vi "VIH HelpGen - Get Control Info - Prepare Name & Description.vi"(9 "Description":string, 11 "Name":string) -> (1 "Description out":string, 3 "Name out":string)   [LabVIEW 2014]
doc: "::: VI Helpeks :::\nCopyright (c) 2000-2026 Konstantin Shifershteyn. All rights reserved."
panel:
  # "VI Helpeks\nCopyright (c) 2012-2026 Konstantin Shifershteyn"
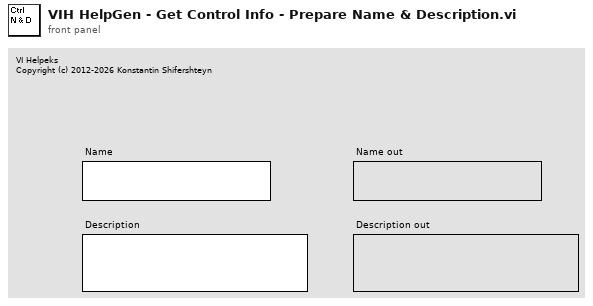
[diagram p1: front panel]
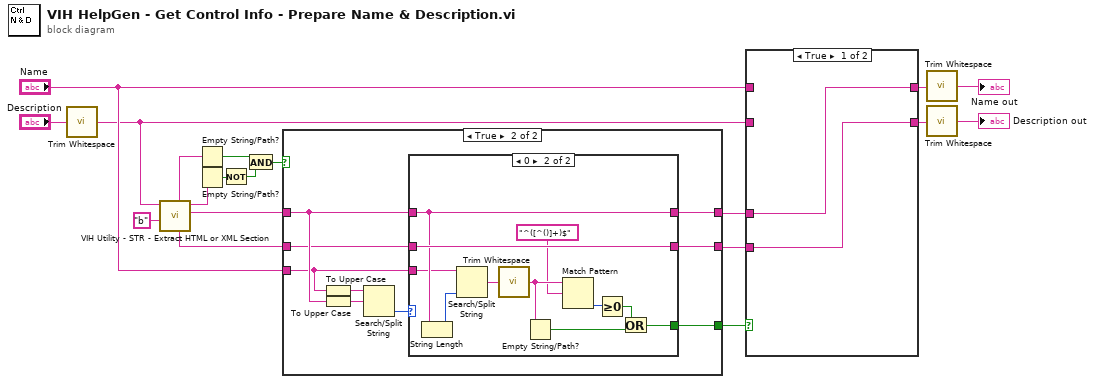
[diagram p0: block diagram]
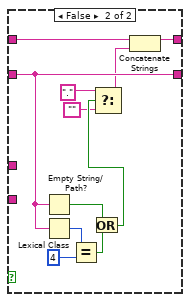
[diagram p2: hidden frame]
diagram:
  n1 = call <vilib>:"Trim Whitespace.vi"("string"="Description") -> ("trimmed string"=w3:string)  [unwired: 1 in]
  n2 = call "VIH Utility - STR - Extract HTML or XML Section.vi"("Section name"="b", "HTML in"=w3) -> ("body"=w11:string, "start"=w14:string, "after"=w10:string, "before"=w17:string)  [unwired: 5 in, 1 out]
  n3 = Empty String/Path?(string/path=w17) -> (empty?=w18:bool)
  n4 = Empty String/Path?(string/path=w14) -> (empty?=w13:bool)
  n5 = Not(x=w13) -> (.not. x?=w12:bool)
  n6 = And(x=w18, y=w12) -> (x .and. y?=w15:bool)
  n7 = case shown="True" w15 {
    tunnel: w11 -> [_ w25]
    tunnel: "Name" -> [_ w21]
    tunnel: [_ w24] -> w7
    tunnel: w10 -> [_ w23]
    tunnel: [_ w22] -> w2
    tunnel: [_ w20] -> w1
    frame False {
    }
    frame True {
      n8 = To Upper Case(1:w21) -> (0:w28:string)
      n9 = To Upper Case(1:w25) -> (0:w27:string)
      n10 = Search/Split String(string=w28, search string/char (-)=w27) -> (offset of match=w26:i32)  [unwired: 1 in, 2 out]
      n11 = case shown="0" w26 {
        tunnel: [_ w38] -> w24
        tunnel: w25 -> [_ w38]
        tunnel: w23 -> [_ w39]
        tunnel: [_ w39] -> w22
        tunnel: w21 -> [_ w37]
        tunnel: [_ w31] -> w20
        frame ..-1, Default {
        }
        frame 0 {
          n12 = String Length(string=w38) -> (length=w36:i32)
          n13 = Search/Split String(string=w37, offset (0)=w36) -> (match + rest of string=w35:string)  [unwired: 1 in, 2 out]
          n14 = call <vilib>:"Trim Whitespace.vi"("string"=w35) -> ("trimmed string"=w30:string)  [unwired: 1 in]
          n15 = Empty String/Path?(string/path=w30) -> (empty?=w34:bool)
          n16 = Match Pattern(string=w30, regular expression="^([^()]+)$") -> (offset past match=w33:i32)  [unwired: 1 in, 3 out]
          n17 = Greater Or Equal To 0?(x=w33) -> (x >= 0?=w32:bool)
          n18 = Or(x=w32, y=w34) -> (x .or. y?=w31:bool)
        }
      }
    }
  }
  n19 = case shown="True" w1 {
    tunnel: [w41 w52] -> w6
    tunnel: w7 -> [w41 _]
    tunnel: w2 -> [w40 _]
    tunnel: [w40 w48] -> w5
    tunnel: "Name" -> [_ w51]
    tunnel: w3 -> [_ w48]
    frame True {
    }
    frame False {
      n20 = Empty String/Path?(string/path=w48) -> (empty?=w47:bool)
      n21 = Lexical Class(1:w48) -> (0:w50:i16)
      n22 = Equal?(x=w50, y=i16 4) -> (x = y?=w46:bool)
      n23 = Or(x=w47, y=w46) -> (x .or. y?=w45:bool)
      n24 = Select(t="." ("string"), s=w45, f="") -> (s? t:f=w42:string)
      n25 = Concatenate Strings(w51, w42) -> (w52:string)
    }
  }
  n26 = call <vilib>:"Trim Whitespace.vi"("string"=w6) -> ("trimmed string"=→"Name out":string)  [unwired: 1 in]
  n27 = call <vilib>:"Trim Whitespace.vi"("string"=w5) -> ("trimmed string"=→"Description out":string)  [unwired: 1 in]
